vi "Ramsete_Execute.vi"(4 "Enabled":bool=TRUE, 6 "Reset":bool, 7 "RAMSETE_EXE_TUNING":T4={"B"=2.0, "Zeta"=0.7, "X Tolerance M"=2.0, "Y Tolerance M"=0.7, "Heading Tolerance RAD"=0.7, "Track Width M"=2.0, "Max Speed M/S"=2.0} {"Max Speed M/S" format="%13.4f"; "Track Width M" format="%13.4f"; "Heading Tolerance RAD" format="%13.4f"; "Y Tolerance M" format="%13.4f"; "X Tolerance M" format="%13.4f"; "Zeta" format="%13.4f"; "B" format="%13.4f"}, 8 "Gyro-Radians\n(Inc counterclockwise)":dbl, 9 "RightDist-Meters":dbl, 10 "LeftDist-Meters":dbl, 11 "TRAJ_STATE":T6 {"POSE"."ROTATION"."SIN" format="%13.4f"; "POSE"."ROTATION"."COS" format="%13.4f"; "POSE"."ROTATION"."VALUE" format="%13.4f"; "POSE"."TRANSLATION"."Y" format="%14.3f"; "POSE"."TRANSLATION"."X" format="%14.3f"}) -> (0 "CurrentRelativePose":T1 {"ROTATION"."SIN" format="%13.4f"; "ROTATION"."COS" format="%13.4f"; "ROTATION"."VALUE" format="%13.4f"; "TRANSLATION"."Y" format="%14.3f"; "TRANSLATION"."X" format="%14.3f"}, 1 "AtReference":bool, 2 "Right Speed Dmd M/S":dbl, 3 "Left Speed Dmd M/S":dbl, 5 "outRAMSETE":T5={"B"=2.0, "Zeta"=0.7, "poseTolerance"={"TRANSLATION"={"X"=0.0, "Y"=0.0}, "ROTATION"={"VALUE"=0.0, "COS"=1.0, "SIN"=0.0}}, "poseError"={"TRANSLATION"={"X"=0.0, "Y"=0.0}, "ROTATION"={"VALUE"=0.0, "COS"=1.0, "SIN"=0.0}}, "Enabled"=TRUE} {"poseError"."ROTATION"."SIN" format="%13.4f"; "poseError"."ROTATION"."COS" format="%13.4f"; "poseError"."ROTATION"."VALUE" format="%13.4f"; "poseError"."TRANSLATION"."Y" format="%14.3f"; "poseError"."TRANSLATION"."X" format="%14.3f"; "poseTolerance"."ROTATION"."SIN" format="%13.4f"; "poseTolerance"."ROTATION"."COS" format="%13.4f"; "poseTolerance"."ROTATION"."VALUE" format="%13.4f"; "poseTolerance"."TRANSLATION"."Y" format="%14.3f"; "poseTolerance"."TRANSLATION"."X" format="%14.3f"; "Zeta" format="%12.3f"; "B" format="%12.3f"})   [LabVIEW 2019, in "Trajectory_Library.lvlib"]
doc: "Convienience function to create and calculate the ramsete control, returning normalized desired left and right speed setpoints \n\nRamsete is a nonlinear time-varying feedback controller for unicycle models that drives the model to a desired pose along a two-dimensional trajectory. Why would we need a nonlinear control law in addition to the linear ones we have used so far like PID? If we use the original approach with PID controllers for left and right position and velocity states, the controllers only deal with the local pose. If the robot deviates from the path, there is no way for the controllers to correct and the robot may not reach the desired global pose. This is due to multiple endpoints existing for the robot which have the same encoder path arc lengths.\n \nInstead of using wheel path arc lengths (which are in the robot's local coordinate frame), nonlinear controllers like pure pursuit and Ramsete use global pose. The controller uses this extra information to guide a linear reference tracker like the PID controllers back in by adjusting the references of the PID controllers.\n\nThe paper \"Control of Wheeled Mobile Robots: An Experimental Overview\" describes a nonlinear controller for a wheeled vehicle with unicycle-like kinematics; a global pose consisting of x, y, and theta; and a desired pose consisting of x_d, y_d, and theta_d. We call it Ramsete because that's the acronym for the title of the book it came from in Italian (\"Robotica Articolata e Mobile per i SErvizi e le TEcnologie\").\n\nParameters: \n - Ramsete EXE Tuning -- Packed data cluster containing the ramsete tuning parameters and Differntial Drive kinematics information.\n - TrajState - Desired trajectory state\n - Left Dist -- The left distance read from encoders (Meters). The encoders do NOT have to be reset at the beginning of trajectory execution.\n - Right Dist -- The right distance read from encoders (Meters). The encoders do NOT have to be reset at the beginning of trajectory execution.\n - Gyro - The current reading of a gyro whose value increases counter clockwise. (You may need to negate your gyro reading.) (Radians)\n - Reset -- Resets the current robot pose and the beginning left and right distances and the gyro reading\n - Enabled -- When enabled uses the ramsete closed loop control to drive the left and right speed demand outputs. When disabled the trajectory data is directly converted to left and right speed demands.\n\n\nReturns:\n - Left Speed Dmd -- Left Speed demand (Meters/Second)\n - Right Speed Dmd -- Right Speed demand (Meters/Second)\n - Out Ramsete -- Updated Ramsete data structure\n - Current Relative Pose -- Current robot relative pose. This pose is reset to zero when the RESET input is set to TRUE. \n - At Reference -- Set to TRUE when the current robot pose is withing the specified tolerance of the desired POSE from the trajectory state input."
uses:
  Trajectory_Library.lvlib
  TypeDef/TRAJ_STATE.ctl
  TypeDef/POSE2D.ctl
  TypeDef/TRANSLATION2D.ctl
  TypeDef/ROTATION2D.ctl
  TypeDef/RAMSETE.ctl
  TypeDef/RAMSETE_EXE_TUNING.ctl
  Translation2d_Create.vi
  <vilib>/Rock Robotics/SystemInterfaces/NetworkCommunication/NetComm_UsageReport_report.vi
  Globals/Util_LibraryGlobals.vi
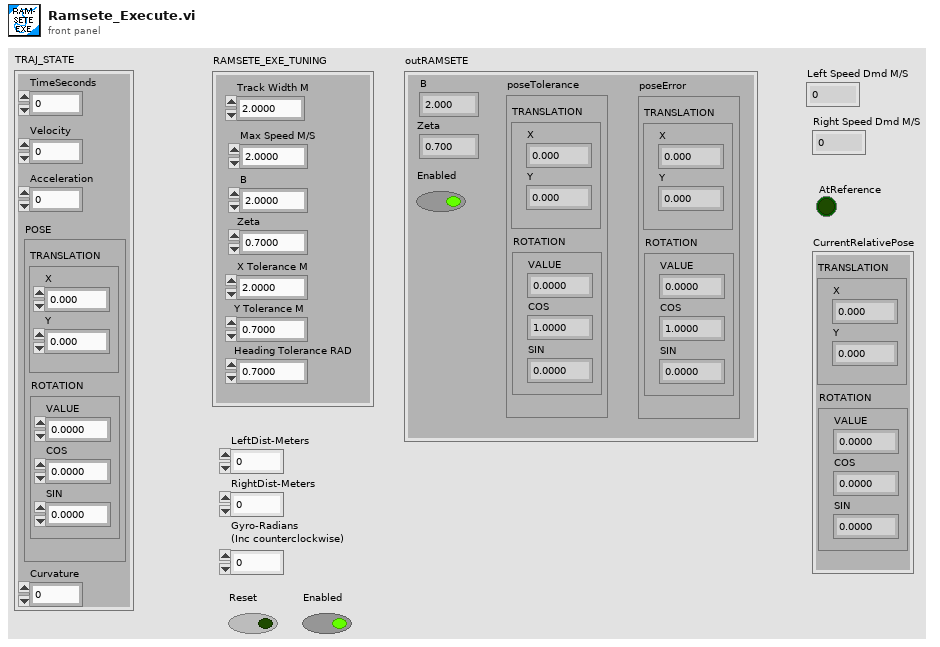
[diagram p1: front panel]
types:
  T1 = typedef "Trajectory_Library.lvlib/POSE2D.ctl" = cluster{"TRANSLATION":T2, "ROTATION":T3}
  T2 = typedef "Trajectory_Library.lvlib/TRANSLATION2D.ctl" = cluster{"X":dbl, "Y":dbl}
  T3 = typedef "Trajectory_Library.lvlib/ROTATION2D.ctl" = cluster{"VALUE":dbl, "COS":dbl, "SIN":dbl}
  T4 = typedef "Trajectory_Library.lvlib/RAMSETE_EXE_TUNING.ctl" = cluster{"B":dbl, "Zeta":dbl, "X Tolerance M":dbl, "Y Tolerance M":dbl, "Heading Tolerance RAD":dbl, "Track Width M":dbl, "Max Speed M/S":dbl}
  T5 = typedef "Trajectory_Library.lvlib/RAMSETE.ctl" = cluster{"B":dbl, "Zeta":dbl, "poseTolerance":T1, "poseError":T1, "Enabled":bool}
  T6 = typedef "Trajectory_Library.lvlib/TRAJ_STATE.ctl" = cluster{"TimeSeconds":dbl, "Velocity":dbl, "Acceleration":dbl, "POSE":T1, "Curvature":dbl}
  T7 = typedef "Trajectory_Library.lvlib/DIFF_DRIVE_KINEMATICS.ctl" = cluster{"TrackWidth_Meters":dbl}
  T8 = typedef "Trajectory_Library.lvlib/CHASSIS_SPEEDS.ctl" = cluster{"vX":dbl, "vY":dbl, "vOmega":dbl}
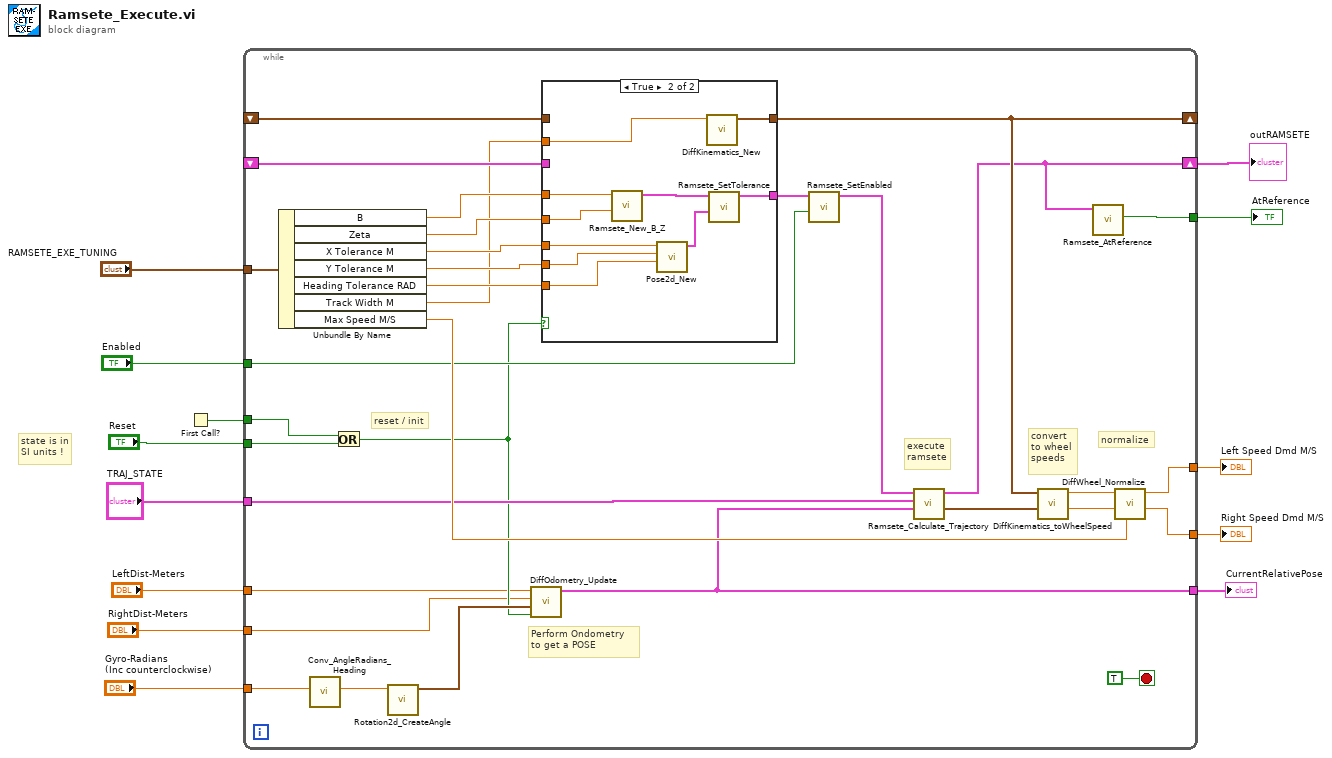
[diagram p0: block diagram]
diagram:
  # "state is in\nSI units !"
  n1 = First Call?() -> (First Call?: T/F=w1:bool)
  n2 = while {
    tunnel: "RAMSETE_EXE_TUNING" -> [w45]
    tunnel: "TRAJ_STATE" -> [w24]
    tunnel: "LeftDist-Meters" -> [w16]
    tunnel: "RightDist-Meters" -> [w15]
    tunnel: [w26] -> w7
    tunnel: [w37] -> w6
    tunnel: [w36] -> w5
    tunnel: "Gyro-Radians\n(Inc counterclockwise)" -> [w35]
    tunnel: "Enabled" -> [w33]
    tunnel: "Reset" -> [w44]
    tunnel: [w27] -> w4
    tunnel: w1 -> [w32]
    shift-right: [w14] -> w11
    shift-left: _ -> [w31]
    shift-right: [w21] -> _
    shift-left: _ -> [w20]
    stop <- TRUE stop-if-true
    # "normalize"
    # "convert\nto wheel\nspeeds"
    # "execute\nramsete"
    # "reset / init"
    # "Perform Ondometry\nto get a POSE"
    n3 = Unbundle By Name(w45) -> ("B"=w43:dbl, "Zeta"=w42:dbl, "X Tolerance M"=w41:dbl, "Y Tolerance M"=w40:dbl, "Heading Tolerance RAD"=w39:dbl, "Track Width M"=w19:dbl, "Max Speed M/S"=w38:dbl)
    n4 = call "Conv_AngleRadians_Heading.vi"("Radians"=w35) -> ("Heading"=w17:dbl)  [unwired: 10 in]
    n5 = Or(x=w32, y=w44) -> (x .or. y?=w18:bool)
    n6 = call "Rotation2d_CreateAngle.vi"("Angle"=w17) -> ("ROTATION"=w29:T3)  [unwired: 10 in]
    n7 = call "DiffOdometry_Update.vi"("Reset"=w18, "Heading"=w29, "RightDistance"=w15, "LeftDistance"=w16) -> ("CurrentRelativePose"=w26:T1)  [unwired: 7 in]
    n8 = case shown="True" w18 {
      tunnel: w43 -> [_ w57]
      tunnel: w42 -> [_ w56]
      tunnel: w41 -> [_ w53]
      tunnel: w40 -> [_ w52]
      tunnel: w39 -> [_ w51]
      tunnel: [w47 w50] -> w34
      tunnel: w31 -> [w47 _]
      tunnel: [w46 w49] -> w21
      tunnel: w19 -> [_ w48]
      tunnel: w20 -> [w46 _]
      frame False {
      }
      frame True {
        n9 = call "Ramsete_New_B_Z.vi"("Zeta"=w56, "B"=w57) -> ("outRAMSETE"=w55:T5)  [unwired: 9 in]
        n10 = call "Pose2d_New.vi"("Heading"=w51, "Y"=w52, "X"=w53) -> ("out POSe"=w54:T1)  [unwired: 8 in]
        n11 = call "DiffKinematics_New.vi"("TrackWidth_Meters"=w48) -> ("DIFF_DRIVE_KINEMATICS"=w49:T7)  [unwired: 10 in]
        n12 = call "Ramsete_SetTolerance.vi"("tolerancePose"=w54, "inRAMSETE"=w55) -> ("outRAMSETE"=w50:T5)  [unwired: 9 in]
      }
    }
    n13 = call "Ramsete_SetEnabled.vi"("Enabled"=w33, "inRAMSETE"=w34) -> ("outRAMSETE"=w25:T5)  [unwired: 9 in]
    n14 = call "Ramsete_Calculate_Trajectory.vi"("CurrentPOSE"=w26, "TRAJ_STATE"=w24, "inRAMSETE"=w25) -> ("CHASSIS Speeds"=w28:T8, "outRAMSETE"=w14:T5)  [unwired: 7 in]
    n15 = call "DiffKinematics_toWheelSpeed.vi"("CHASSIS Speed"=w28, "DIFF_DRIVE_KINEMATICS"=w21) -> ("RightVelocity"=w22:dbl, "LeftVelocity"=w23:dbl)  [unwired: 8 in]
    n16 = call "Ramsete_AtReference.vi"("RAMSETE"=w14) -> ("AtReference"=w27:bool)  [unwired: 10 in]
    n17 = call "DiffWheel_Normalize.vi"("Max Speed"=w38, "Right Wheel Demand"=w22, "Left Wheel Demand"=w23) -> ("Normalized Right Wheel Demand"=w36:dbl, "Normalized Left Wheel Demand"=w37:dbl)  [unwired: 7 in]
  }
  "outRAMSETE" <- w11
  "CurrentRelativePose" <- w7
  "Left Speed Dmd M/S" <- w6
  "Right Speed Dmd M/S" <- w5
  "AtReference" <- w4
